vi "Create.vi"(7 "Direction":T1, 8 "error in (no error)":errorcluster, 9 "Custom Config Data":u8[](array[numeric]), 10 "Name":string, 11 "CIF_Iceoryx_BB in":refnum<class "CIF_Iceoryx_BB.lvclass">) -> (0 "error out":errorcluster, 3 "CIF_Iceoryx_BB out":refnum<class "CIF_Iceoryx_BB.lvclass">)   [LabVIEW 2021, in "CIF_Iceoryx_BB.lvclass"]
uses:
  CIF_Iceoryx_BB.lvclass
  D:/dev/Packages/CIF_Channels_Core/src/CIFChannels/CIFChannels.lvclass
  ChannelCommon/typedef/Direction.ctl
  <vilib>/CIF Foundation/CIF Iceoryx/typedef/Topic Full Names.ctl
  ChannelCommon/typedef/Disconnect Behavior.ctl
  ChannelCommon/typedef/Channel Pattern.ctl
  CIF_Iceoryx_BB.lvclass/CIF_Iceoryx_BB.ctl
  ChannelCommon/typedef/Channel State.ctl
  CIFChannels/CIFChannels.lvclass/CIFChannels.ctl
  Accessors/Write Writer Reference.vi
  Accessors/Write Data Configuration.vi
  CIFChannels/Accessors/Write Pattern.vi
  CIFChannels/Accessors/Write Channel State.vi
  Accessors/Read Blackboard Reference.vi
  ChannelCommon/ChannelCommon.lvlib
  <vilib>/CIF Foundation/CIF Iceoryx/Iceoryx.lvlib
  CIFChannels/CIFChannels.lvclass
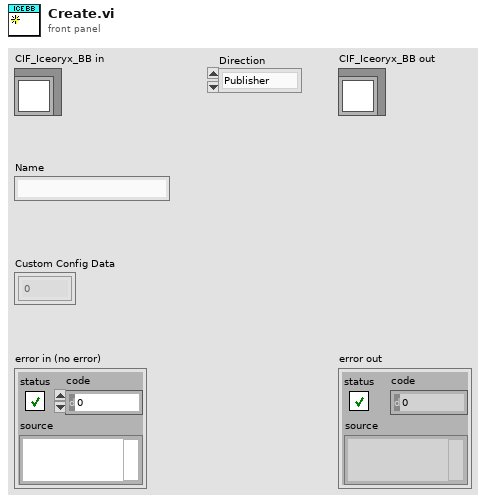
[diagram p1: front panel]
types:
  T1 = typedef "ChannelCommon.lvlib/Direction.ctl" = enum8{"Publisher", "Subscriber"}
  T2 = typedef "Iceoryx.lvlib/Topic Full Names.ctl" = cluster{"BlackBoard":string, "Topic":string, "Type Override":string}
  T3 = typedef "ChannelCommon.lvlib/Disconnect Behavior.ctl" = enum8{"Default value", "Last value", "Error with default"}
  T4 = typedef "ChannelCommon.lvlib/Channel Pattern.ctl" = enum8{"Unknown", "Tag", "FIFO", "MultiFIFO", "BackpressureFIFO"}
  T5 = typedef "ChannelCommon.lvlib/Channel State.ctl" = enum8{"Creating", "Disconnected", "Connecting", "Connected", "Destroyed"}
  T6 = typedef "Iceoryx.lvlib/BB Refnum.ctl" = cluster{"refnum":u64, "BB":enum8{"bb"}}
  T7 = typedef "Iceoryx.lvlib/BB Writer Refnum.ctl" = cluster{"refnum":u64, "BB Writer":enum8{"bb_writer"}}
  T8 = typedef "CIF_Iceoryx_BB.lvclass/Data Configuration.ctl" = cluster{"Element Size":u32, "Element Alignment":u32, "Array":bool, "Type":string}
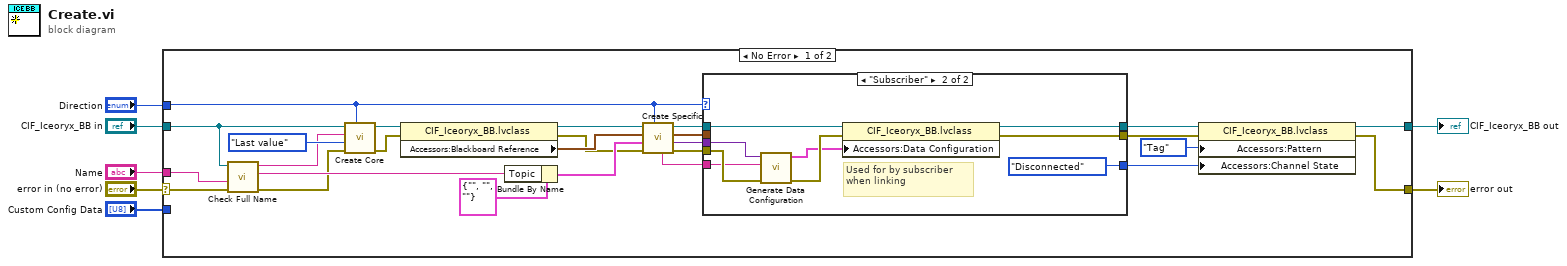
[diagram p0: block diagram]
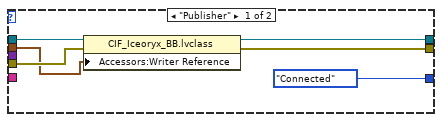
[diagram p2: hidden frame]
diagram:
  n1 = case shown="No Error" "error in (no error)" {
    selector: "error in (no error)" -> [w24 w50]
    tunnel: [w33 w50] -> w2
    tunnel: [w32 w49] -> w3
    tunnel: "CIF_Iceoryx_BB in" -> [w28 w49]
    tunnel: "Name" -> [w27 _]
    tunnel: "Direction" -> [w9 _]
    tunnel: "Custom Config Data" -> [_ _]
    frame No Error {
      n2 = call "Check Full Name.vi"("error in (no error)"=w24, "Topic Name In"=w27, "CIF_Iceoryx_BB in"=w28) -> ("error out"=w23:errorcluster, "Topic Name out"=w25:string, "Full Name Out"=w26:string)  [unwired: 6 in]
      n3 = call "Create Core.vi"("Direction"=w9, "error in (no error)"=w23, "Disconnect Behavior"=Disconnect_Behavior."Last value", "Name"=w26, "CIFChannels in"=w28) -> ("error out"=w18:errorcluster, "CIFChannels out"=w29:refnum<class "CIF_Iceoryx_BB.lvclass">)  [unwired: 2 in, 3 out]
      n4 = property class="CIF_Iceoryx_BB.lvclass"(reference=w29, error in=w18) -> (reference out=w19:refnum<class "CIF_Iceoryx_BB.lvclass">, error out=w17:errorcluster, "Accessors:Blackboard Reference"=w20:T6)
      n5 = Bundle By Name(cluster=T2 {"BlackBoard"="", "Topic"="", "Type Override"=""} ("Topic Name"), "Topic"=w25) -> (w21:T2)
      n6 = call-dynamic "Create Specific.vi"("Direction"=w9, "error in (no error)"=w17, "Topic Name"=w21, "Blackboard Reference"=w20, "CIF_Iceoryx_BB in"=w19) -> ("error out"=w14:errorcluster, "Data Variant"=w15:variant, "Writer Reference"=w13:T7, "CIF_Iceoryx_BB out"=w16:refnum<class "CIF_Iceoryx_BB.lvclass">, "Cluster or Array String"=w8:string)  [unwired: 2 in]
      n7 = case shown="\"Subscriber\"" w9 {
        tunnel: [Channel_State."Connected" ("Channel State") Channel_State."Disconnected" ("Channel State")] -> w10
        tunnel: [w38 w47] -> w11
        tunnel: w16 -> [w37 w46]
        tunnel: w15 -> [_ w45]
        tunnel: w14 -> [w36 w44]
        tunnel: w13 -> [w35 _]
        tunnel: [w34 w43] -> w12
        tunnel: w8 -> [_ w41]
        frame "Publisher" {
          n8 = property class="CIF_Iceoryx_BB.lvclass"(reference=w37, error in=w36, "Accessors:Writer Reference"=w35) -> (reference out=w38:refnum<class "CIF_Iceoryx_BB.lvclass">, error out=w34:errorcluster)
        }
        frame "Subscriber" {
          # "Used for by subscriber when linking"
          n9 = call "Generate Data Configuration.vi"("error in (no error)"=w44, "Cluster or Array String"=w41, "Data"=w45) -> ("error out"=w42:errorcluster, "Data Configuration"=w40:T8)  [unwired: 7 in]
          n10 = property class="CIF_Iceoryx_BB.lvclass"(reference=w46, error in=w42, "Accessors:Data Configuration"=w40) -> (reference out=w47:refnum<class "CIF_Iceoryx_BB.lvclass">, error out=w43:errorcluster)
        }
      }
      n11 = property class="CIF_Iceoryx_BB.lvclass"(reference=w11, error in=w12, "Accessors:Pattern"=Channel_Pattern."Tag" ("Pattern"), "Accessors:Channel State"=w10) -> (reference out=w32:refnum<class "CIF_Iceoryx_BB.lvclass">, error out=w33:errorcluster)
    }
    frame Error {
    }
  }
  "error out" <- w2
  "CIF_Iceoryx_BB out" <- w3
